vi "Make.vi"() -> ()   [LabVIEW 2019]
doc: "Quick and dirty makefile."
uses:
  <vilib>/AppBuilder/AB_API_Simple/Build (path).vi
  <vilib>/AppBuilder/AB_API_Simple/NI_App_Builder_API.lvlib
panel:
  out "error out":errorcluster
  out "Currently building":path
  out "Generated files":path[](array[path])
  # "Note: Ensure all projects are closed in memory, then run this VI."
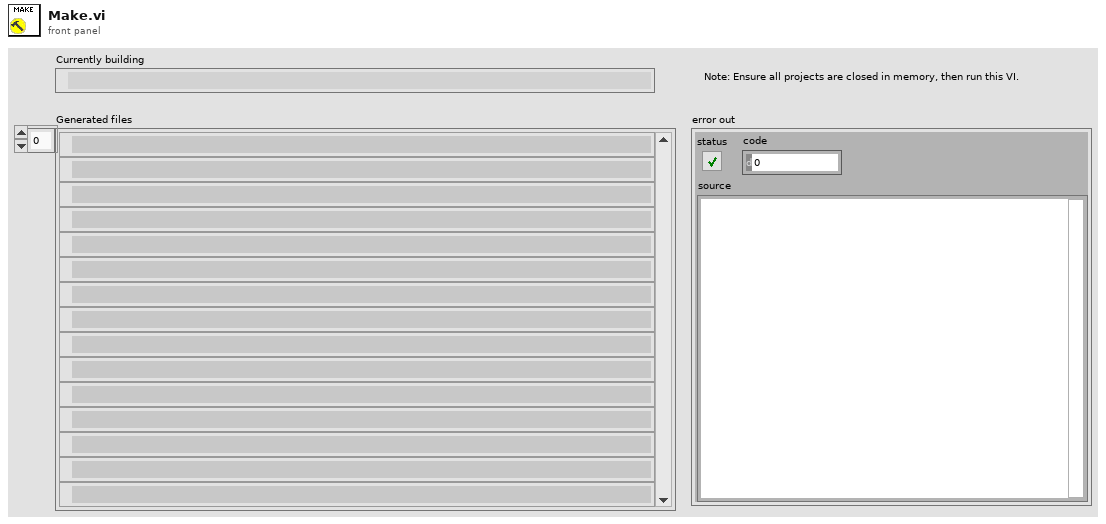
[diagram p1: front panel]
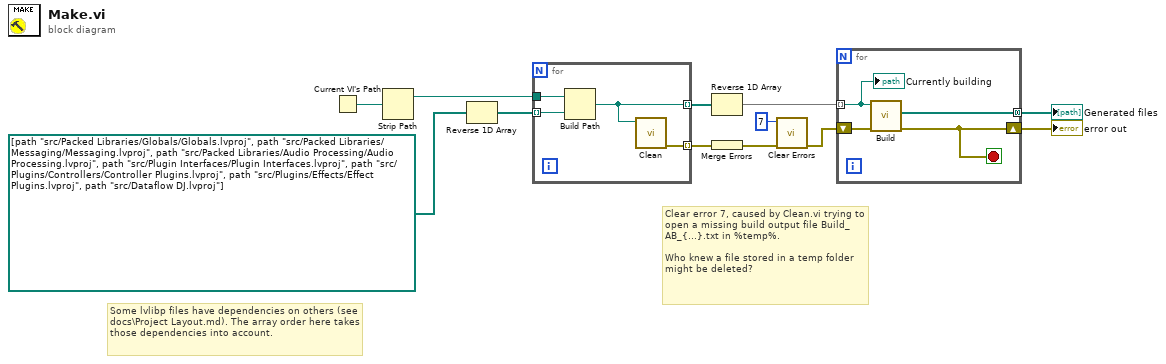
[diagram p0: block diagram]
diagram:
  # "Clear error 7, caused by Clean.vi trying to open a missing build output file Build_AB_{...}.txt in %temp%.\n\nWho knew a file stored in a temp folder might be deleted?"
  # "Some lvlibp files have dependencies on others (see docs\\Project Layout.md). The array order here takes those dependencies into account."
  n1 = Current VI's Path() -> (path=w12:path)
  n2 = Strip Path(path=w12) -> (stripped path=w10:path)  [unwired: 1 out]
  n3 = Reverse 1D Array(array=path[] [path "src/Packed Libraries/Globals/Globals.lvproj", path "src/Packed Libraries/Messaging/Messaging.lvproj", path "src/Packed Libraries/Audio Processing/Audio Processing.lvproj", path "src/Plugin Interfaces/Plugin Interfaces.lvproj", path "src/Plugins/Controllers/Controller Plugins.lvproj", path "src/Plugins/Effects/Effect Plugins.lvproj", path "src/Dataflow DJ.lvproj"]) -> (reversed array=w2:path[])
  n4 = for {
    tunnel: w2 -> [w16] mode=indexing
    tunnel: w10 -> [w15]
    tunnel: [w14] -> w7 mode=indexing
    tunnel: [w13] -> w6 mode=indexing
    n5 = Build Path(base path=w15, name or relative path=w16) -> (appended path=w14:path)
    n6 = call <vilib>:"Clean.vi"("Path to project"=w14) -> ("error out"=w13:errorcluster)  [unwired: 10 in]
  }
  n7 = Reverse 1D Array(array=w7) -> (reversed array=w1:path[])
  n8 = Merge Errors(w6) -> (w5:errorcluster)
  n9 = call <vilib>:"Clear Errors.vi"("error in (no error)"=w5, "specific error code to clear (0: all)"=7) -> ("error out"=w3:errorcluster)  [unwired: 4 in, 1 out]
  n10 = for {
    tunnel: [w20] -> w9 mode=concatenating
    tunnel: w1 -> [w19] mode=indexing
    shift-right: [w18] -> w8
    shift-left: w3 -> [w17]
    stop <- w18 stop-if-true
    n11 = call-poly <vilib>:"Build.vi"("error in (no error)"=w17, "Path to project"=w19) -> ("error out"=w18:errorcluster, "Generated files"=w20:path[])  [unwired: 8 in]
    "Currently building" <- w19
  }
  "Generated files" <- w9
  "error out" <- w8
